vi "ADT760.vi"(4 "Error In":errorcluster, 7 "Command":string) -> (0 "Error Out":errorcluster, 3 "Response":string)   [LabVIEW 2018]
uses:
  MOKO_LabViewLibrary/MokoLowLevel/MokoLowLovelControl/MLLC_ConnectCluster.ctl
  MOKO_LabViewLibrary/MokoLowLevel/MokoLowLovelControl/MLLC_InterfaceType.ctl
  MOKO_LabViewLibrary/MokoLowLevel/MokoLowLovelControl/MLLC_OpenedSession.ctl
  MOKO_LabViewLibrary/MokoLowLevel/MokoLowLovelControl/MLLC_InterfaceSettings.ctl
  MOKO_LabViewLibrary/MokoLowLevel/MokoLowLovelControl/MLLC_InterfaceKind.ctl
panel:
  in  "ResponseInit":string="ADT760"
  in  "Request":string="*IDN?"
  in  "Settings":cluster{"Connect":T1, "PressureModule":string}={"Connect"={"InterfaceType"=enum."VISA", "OpenedSession"="", "InterfaceSettings"={"Interface"=enum."RS232", "EOS 4 read"=enum."LF (\\n)", "EOS 4 write"=enum."LF (\\n)", "TMO, ms"=10000, "Sett"=variant(cluster{"Baud Rate":u32, "Data Bits":u16, "Parity":u16, "Stop Bits":u16, "Flow Control":u16, "Eho":bool} {"Baud Rate"=75, "Data Bits"=0, "Parity"=0, "Stop Bits"=0, "Flow Control"=0, "Eho"=FALSE})}}, "PressureModule"="1"}
  in  "Error Code":u32
  in  "Driver Name":string="ADT760"
  in  "Mode":T6(ring)=enum."Check"
  # "ADT760"
  # "20"
  # "B7"
  # "A0"
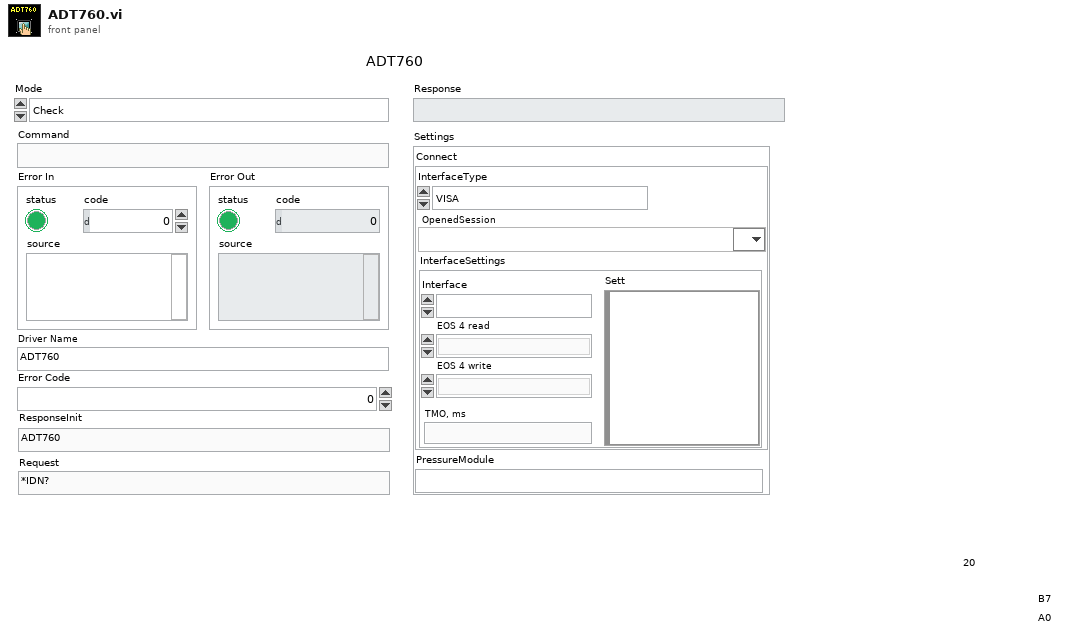
[diagram p1: front panel]
types:
  T1 = typedef "MLLC_ConnectCluster.ctl" = cluster{"InterfaceType":T2, "OpenedSession":T3, "InterfaceSettings":T4}
  T2 = typedef "MLLC_InterfaceType.ctl" = enum16{"VISA", "Prologix USB-GPIB"}
  T3 = typedef "MLLC_OpenedSession.ctl" = refnum<visa-resource-name>
  T4 = typedef "MLLC_InterfaceSettings.ctl" = cluster{"Interface":T5, "EOS 4 read":enum16{"Default (=EOS 4 write)", "CR (\\r)", "LF (\\n)", "None"}, "EOS 4 write":enum16{"CR+LF (\\r\\n)", "CR (\\r)", "LF (\\n)", "None"}, "TMO, ms":i32, "Sett":variant}
  T5 = typedef "MLLC_InterfaceKind.ctl" = enum16{"RS232", "GPIB", "USB", "Ethernet", "another"}
  T6 = enum16{"get", "set", "close", "Init", "Check", "ID"}
  T7 = typedef "MLLC_Mode.ctl" = enum16{"get", "set", "close", "Init", "Check"}
  T8 = typedef "MLLC_Error.ctl" = errorcluster
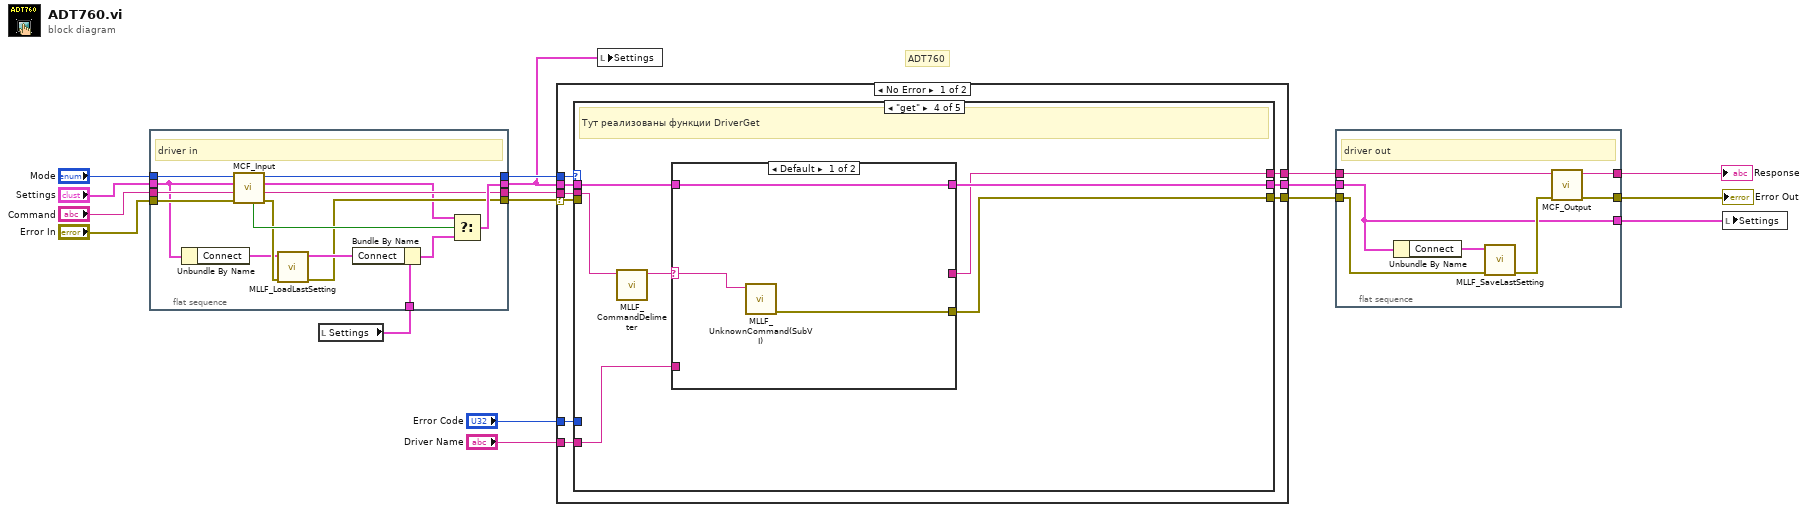
[diagram p0: block diagram]
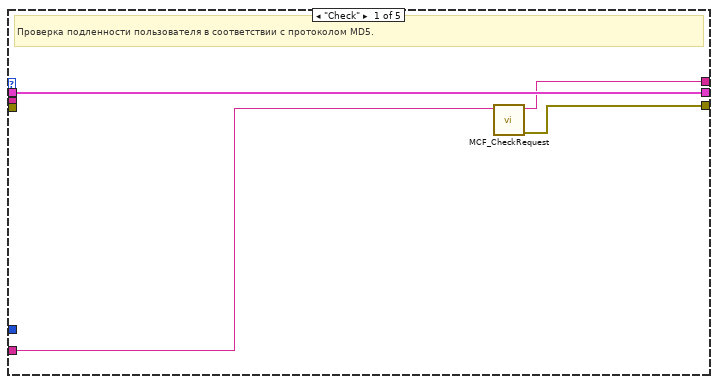
[diagram p2: hidden frame]
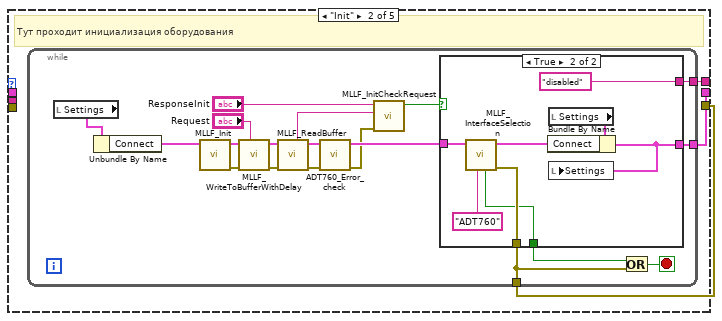
[diagram p3: hidden frame]
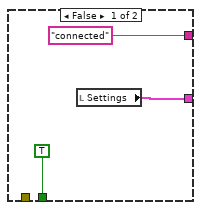
[diagram p4: hidden frame]
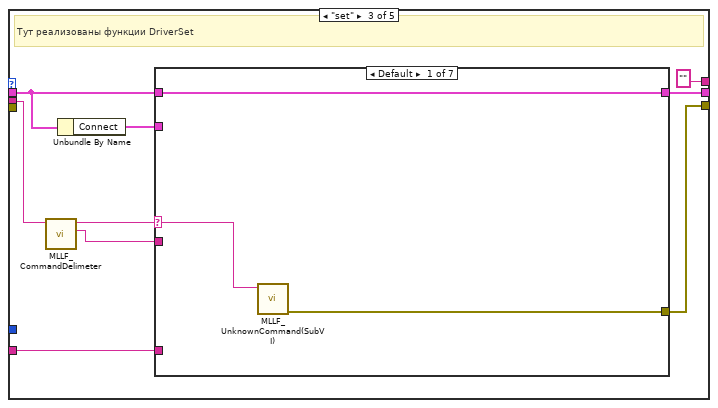
[diagram p5: hidden frame]
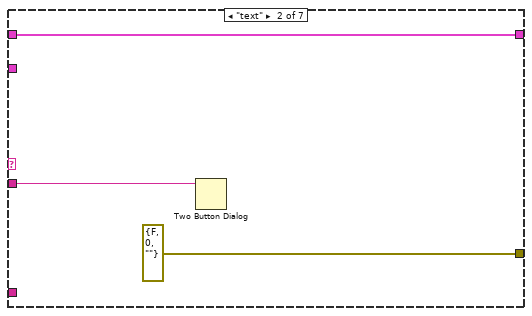
[diagram p6: hidden frame]
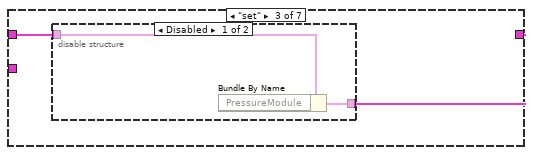
[diagram p7: hidden frame]
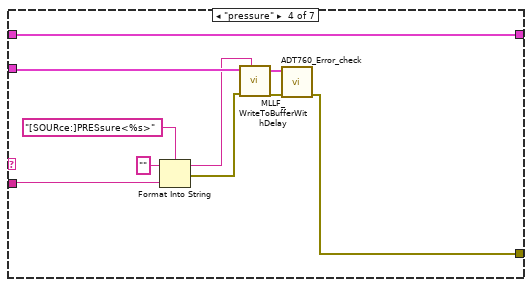
[diagram p9: hidden frame]
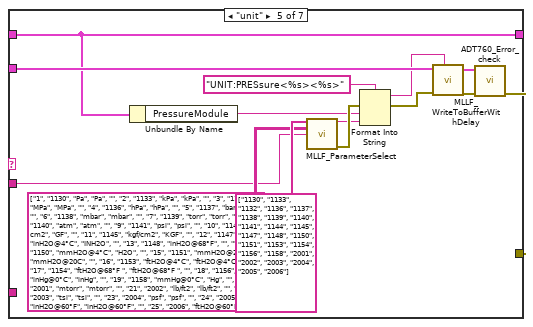
[diagram p10: hidden frame]
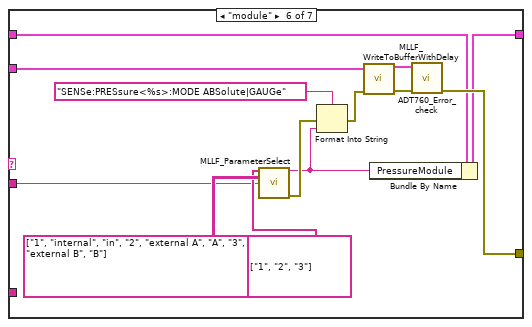
[diagram p11: hidden frame]
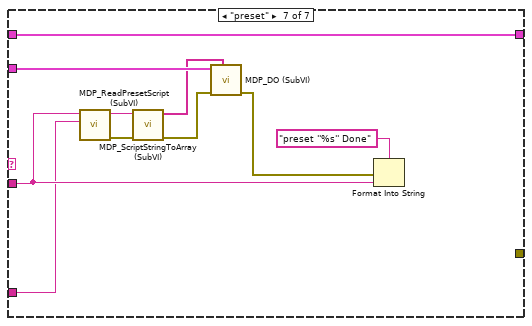
[diagram p12: hidden frame]
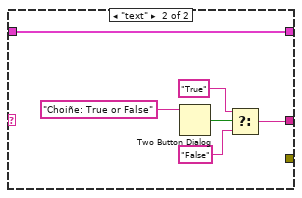
[diagram p13: hidden frame]
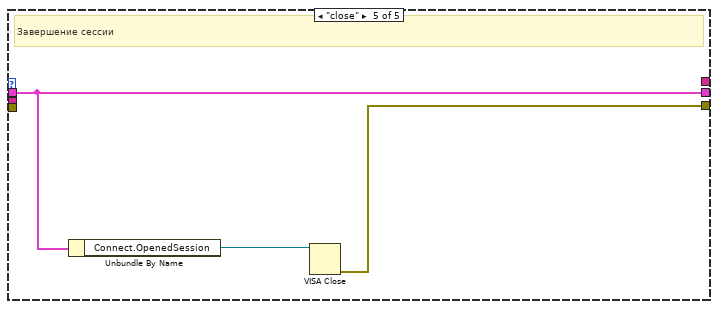
[diagram p14: hidden frame]
diagram:
  # "ADT760"
  n1 = flat-sequence {
    tunnel: [w22] -> w8
    tunnel: [w24] -> w7
    tunnel: "Command" -> [w25]
    tunnel: "Mode" -> [w27]
    tunnel: "Settings" -> [w19]
    tunnel: [w29] -> w10
    tunnel: w9 -> [w28]
    tunnel: "Error In" -> [w21]
    tunnel: [w20] -> w11
    frame #0 {
      # "driver in"
      n2 = Unbundle By Name(w19) -> ("Connect"=w18:T1)
      n3 = call "MCF_Input.vi"("error in (no error)"=w21, "Command"=w25, "Mode"=w27) -> ("error out"=w23:errorcluster, "Command out"=w24:string, "Mode out"=w20:T7, "Boolean"=w26:bool)  [unwired: 5 in]
      n4 = call "MLLF_LoadLastSetting.vi"("Error In"=w23, "DriverConnectCluster in"=w18) -> ("Error Out"=w22:errorcluster, "DriverConnectCluster out"=w30:T1)  [unwired: 8 in]
      n5 = Bundle By Name(cluster=w28, "Connect"=w30) -> (w31:cluster{"Connect":T1, "PressureModule":string})
      n6 = Select(t=w19, s=w26, f=w31) -> (s? t:f=w29:cluster{"Connect":T1, "PressureModule":string})
    }
  }
  n7 = local read "Settings"() -> (w9:cluster{"Connect":T1, "PressureModule":string})
  n8 = case shown="No Error" w8 {
    selector: w8 -> [w36 w164]
    tunnel: [w38 w164] -> w4
    tunnel: w11 -> [w40 _]
    tunnel: [w39 _] -> w6
    tunnel: w7 -> [w37 _]
    tunnel: w10 -> [w33 w163]
    tunnel: "Error Code" -> [w35 _]
    tunnel: "Driver Name" -> [w34 _]
    tunnel: [w32 w163] -> w5
    frame No Error {
      n9 = case shown="\"get\"" w40 {
        tunnel: [w42 w46 "" ("Output String") w148 _] -> w39
        tunnel: [w41 w45 w81 w147 w161] -> w38
        tunnel: w37 -> [_ _ w80 w145 _]
        tunnel: w36 -> [_ _ _ _ _]
        tunnel: w35 -> [_ _ _ _ _]
        tunnel: w34 -> [w43 _ w84 w144 _]
        tunnel: w33 -> [w44 _ w86 w150 w160]
        tunnel: [w44 w47 w85 w149 w160] -> w32
        frame "Check" {
          # "Проверка подленности пользователя в соответствии с протоколом MD5."
          n10 = call "MCF_CheckRequest.vi"("Driver Name"=w43) -> ("Error Out"=w41:errorcluster, "Output String"=w42:string)  [unwired: 9 in]
        }
        frame "Init" {
          # "Тут проходит инициализация оборудования"
          n11 = while {
            tunnel: [w63] -> w47
            tunnel: [w49] -> w46
            tunnel: [w48] -> w45
            stop <- w65 stop-if-true
            n12 = local read "Settings"() -> (w64:cluster{"Connect":T1, "PressureModule":string})
            n13 = Unbundle By Name(w64) -> ("Connect"=w62:T1)
            n14 = call "MLLF_Init.vi"("DriverConnect in"=w62) -> ("Error Out"=w54:errorcluster, "DriverConnect out"=w55:T1)  [unwired: 7 in]
            n15 = call "MLLF_WriteToBufferWithDelay.vi"("Command"="Request", "Error In"=w54, "DriverConnect in"=w55) -> ("Error Out"=w61:errorcluster, "DriverConnect out"=w60:T1)  [unwired: 7 in]
            n16 = call "MLLF_ReadBuffer.vi"("Error In"=w61, "DriverConnect in"=w60) -> ("Error Out"=w58:errorcluster, "DriverConnect out"=w59:T1, "String"=w52:string)  [unwired: 6 in]
            n17 = call "ADT760_Error_check.vi"("Error In"=w58, "DriverConnect in"=w59) -> ("Error Out"=w51:errorcluster, "DriverConnect out"=w56:T1)  [unwired: 8 in]
            n18 = call "MLLF_InitCheckRequest.vi"("error in (no error)"=w51, "Answer"=w52, "Response Init"="ResponseInit") -> ("Design"=w50:bool)  [unwired: 5 in, 3 out]
            n19 = case shown="True" w50 {
              tunnel: w56 -> [_ w76]
              tunnel: [TRUE w71] -> w66
              tunnel: [_ w77] -> w48
              tunnel: [w68 w72] -> w63
              tunnel: ["connected" "disabled"] -> w49
              frame False {
                n20 = local read "Settings"() -> (w68:cluster{"Connect":T1, "PressureModule":string})
              }
              frame True {
                n21 = call "MLLF_InterfaceSelection.vi"("Driver Name"="ADT760" ("String"), "DriverConnect in"=w76) -> ("error out"=w77:T8, "DriverConnect out"=w74:T1, "stop init?"=w71:bool)  [unwired: 7 in]
                n22 = local read "Settings"() -> (w73:cluster{"Connect":T1, "PressureModule":string})
                n23 = Bundle By Name(cluster=w73, "Connect"=w74) -> (w72:cluster{"Connect":T1, "PressureModule":string})
                n24 = local write "Settings"(w72) -> ()
              }
            }
            n25 = Or(x=w66, y=w48) -> (x .or. y?=w65:bool)
          }
        }
        frame "set" {
          # "Тут реализованы функции DriverSet"
          n26 = call "MLLF_CommandDelimeter.vi"("command with param"=w80) -> ("param 1"=w78:string, "command"=w79:string)  [unwired: 6 in, 3 out]
          n27 = Unbundle By Name(w86) -> ("Connect"=w82:T1)
          n28 = case shown="Default" w79 {
            selector: w79 -> [w88 _ _ _ _ _ _]
            tunnel: [w89 w92 w93 w102 w111 w128 w134] -> w85
            tunnel: w86 -> [w89 w92 w94 w102 w111 w129 w134]
            tunnel: w82 -> [_ _ _ w104 w117 w127 w138]
            tunnel: w78 -> [_ w90 _ w97 w110 w130 w137]
            tunnel: [w87 errorcluster {"status"=FALSE, "code"=0, "source"=""} ("error IO") _ w98 w116 w133 _] -> w81
            tunnel: w84 -> [_ _ _ _ _ _ w136]
            frame Default {
              n29 = call "MLLF_UnknownCommand(SubVI).vi"("Unknown command"=w88) -> ("error out"=w87:errorcluster)  [unwired: 10 in]
            }
            frame "text" {
              n30 = Two Button Dialog(message=w90) -> ()  [unwired: 2 in, 1 out]
            }
            frame "set" {
              n31 = disable-structure shown="Disabled" {
                disable-tunnel: w94 -> [w96 _]
                disable-tunnel: [w95 _] -> w93
                frame Disabled {
                  n32 = Bundle By Name(cluster=w96) -> (w95:cluster{"Connect":T1, "PressureModule":string})  [unwired: 1 in]
                }
                frame Enabled {
                }
              }
            }
            frame "pressure" {
              n33 = Format Into String(format string="[SOURce:]PRESsure<%s>", initial string="", w97) -> (resulting string=w103:string, error out=w101:errorcluster)  [unwired: 1 in]
              n34 = call "MLLF_WriteToBufferWithDelay.vi"("Command"=w103, "Error In"=w101, "DriverConnect in"=w104) -> ("Error Out"=w99:errorcluster, "DriverConnect out"=w100:T1)  [unwired: 7 in]
              n35 = call "ADT760_Error_check.vi"("Error In"=w99, "DriverConnect in"=w100) -> ("Error Out"=w98:errorcluster)  [unwired: 8 in, 1 out]
            }
            frame "unit" {
              n36 = Unbundle By Name(w111) -> ("PressureModule"=w112:string)
              n37 = call "MLLF_ParameterSelect.vi"("Command to equipment"=string[] ["1130", "1133", "1132", "1136", "1137", "1138", "1139", "1140", "1141", "1144", "1145", "1147", "1148", "1150", "1151", "1153", "1154", "1156", "1158", "2001", "2002", "2003", "2004", "2005", "2006"] ("Command 2 equipment"), "Names"=string[][] [["1", "1130", "Pa", "Pa", ""], ["2", "1133", "kPa", "kPa", ""], ["3", "1132", "MPa", "MPa", ""], ["4", "1136", "hPa", "hPa", ""], ["5", "1137", "bar", "bar", ""], ["6", "1138", "mbar", "mbar", ""], ["7", "1139", "torr", "torr", ""], ["8", "1140", "atm", "atm", ""], ["9", "1141", "psi", "psi", ""], ["10", "1144", "gf/cm2", "GF", ""], ["11", "1145", "kgf/cm2", "KGF", ""], ["12", "1147", "inH2O@4°C", "INH2O", ""], ["13", "1148", "inH2O@68°F", "", ""], ["14", "1150", "mmH2O@4°C", "H2O", ""], ["15", "1151", "mmH2O@20°C ", "mmH2O@20C", ""], ["16", "1153", "ftH2O@4°C", "ftH2O@4°C", ""], ["17", "1154", "ftH2O@68°F ", "ftH2O@68°F ", ""], ["18", "1156", "inHg@0°C", "inHg", ""], ["19", "1158", "mmHg@0°C", "Hg", ""], ["20", "2001", "mtorr", "mtorr", ""], ["21", "2002", "lb/ft2", "lb/ft2", ""], ["22", "2003", "tsi", "tsi", ""], ["23", "2004", "psf", "psf", ""], ["24", "2005", "inH2O@60°F", "inH2O@60°F", ""], ["25", "2006", "ftH2O@60°F ", "ftH2O@60°F ", ""]], "Input"=w110) -> ("Choice"=w109:string, "Error Out"=w120:errorcluster)  [unwired: 11 in]
              n38 = Format Into String(format string="UNIT:PRESsure<%s><%s>", error in=w120, w112, w109) -> (resulting string=w108:string, error out=w107:errorcluster)  [unwired: 1 in]
              n39 = call "MLLF_WriteToBufferWithDelay.vi"("Command"=w108, "Error In"=w107, "DriverConnect in"=w117) -> ("Error Out"=w118:errorcluster, "DriverConnect out"=w119:T1)  [unwired: 7 in]
              n40 = call "ADT760_Error_check.vi"("Error In"=w118, "DriverConnect in"=w119) -> ("Error Out"=w116:errorcluster)  [unwired: 8 in, 1 out]
            }
            frame "module" {
              n41 = call "MLLF_ParameterSelect.vi"("Command to equipment"=string[] ["1", "2", "3"] ("Command 2 equipment"), "Names"=string[][] [["1", "internal", "in"], ["2", "external A", "A"], ["3", "external B", "B"]], "Input"=w130) -> ("Choice"=w123:string, "Error Out"=w126:errorcluster)  [unwired: 11 in]
              n42 = Format Into String(format string="SENSe:PRESsure<%s>:MODE ABSolute|GAUGe", error in=w126, w123) -> (error out=w125:errorcluster)  [unwired: 1 in, 1 out]
              n43 = call "MLLF_WriteToBufferWithDelay.vi"("Error In"=w125, "DriverConnect in"=w127) -> ("Error Out"=w121:errorcluster, "DriverConnect out"=w122:T1)  [unwired: 8 in]
              n44 = Bundle By Name(cluster=w129, "PressureModule"=w123) -> (w128:cluster{"Connect":T1, "PressureModule":string})
              n45 = call "ADT760_Error_check.vi"("Error In"=w121, "DriverConnect in"=w122) -> ("Error Out"=w133:errorcluster)  [unwired: 8 in, 1 out]
            }
            frame "preset" {
              n46 = call "MDP_ReadPresetScript (SubVI).vi"("Driver Name"=w136, "String in"=w137) -> ("Error Out"=w141:errorcluster, "String out"=w142:string)  [unwired: 8 in]
              n47 = call "MDP_ScriptStringToArray (SubVI).vi"("Error In"=w141, "String script"=w142) -> ("Error Out"=w143:errorcluster, "Array script"=w135:string[])  [unwired: 8 in]
              n48 = call "MDP_DO (SubVI).vi"("Array script"=w135, "Error in (no error)"=w143, "DriverConnect in"=w138) -> ("Error Out"=w139:errorcluster)  [unwired: 7 in, 1 out]
              n49 = Format Into String(format string="preset ''%s'' Done" ("Befor substring"), error in=w139, w137) -> ()  [unwired: 1 in, 2 out]
            }
          }
        }
        frame "get" {
          # "Тут реализованы функции DriverGet"
          n50 = call "MLLF_CommandDelimeter.vi"("command with param"=w145) -> ("command"=w146:string)  [unwired: 6 in, 4 out]
          n51 = case shown="Default" w146 {
            selector: w146 -> [w152 _]
            tunnel: w150 -> [w153 w159]
            tunnel: [w153 w159] -> w149
            tunnel: [_ w154] -> w148
            tunnel: [w151 _] -> w147
            tunnel: w144 -> [_ _]
            frame Default {
              n52 = call "MLLF_UnknownCommand(SubVI).vi"("Unknown command"=w152) -> ("error out"=w151:errorcluster)  [unwired: 10 in]
            }
            frame "text" {
              n53 = Two Button Dialog(message="Choiñe: True or False") -> (T button?=w158:bool)  [unwired: 2 in]
              n54 = Select(t="True" ("string"), s=w158, f="False" ("string")) -> (s? t:f=w154:string)
            }
          }
        }
        frame "close" {
          # "Завершение сессии"
          n55 = Unbundle By Name(w160) -> ("Connect.OpenedSession"=w162:T3)
          n56 = VISA Close(VISA resource name=w162) -> (error out=w161:errorcluster)  [unwired: 1 in]
        }
      }
    }
    frame Error {
    }
  }
  n57 = local write "Settings"(w10) -> ()
  n58 = flat-sequence {
    tunnel: [w171] -> w3
    tunnel: w6 -> [w170]
    tunnel: w4 -> [w166]
    tunnel: w5 -> [w167]
    tunnel: [w167] -> w1
    tunnel: [w168] -> w2
    frame #0 {
      # "driver out"
      n59 = Unbundle By Name(w167) -> ("Connect"=w165:T1)
      n60 = call "MLLF_SaveLastSetting.vi"("error in"=w166, "DriverConnectCluster in"=w165) -> ("error out"=w169:T8)  [unwired: 8 in, 1 out]
      n61 = call "MCF_Output.vi"("Error In"=w169, "Input"=w170) -> ("Error Out"=w168:errorcluster, "Output"=w171:string)  [unwired: 8 in]
    }
  }
  n62 = local write "Settings"(w1) -> ()
  "Response" <- w3
  "Error Out" <- w2
